vi "Perfect Number Check.vi"() -> ()   [LabVIEW 2026]
panel:
  out "Sum of Divisors":dbl
  out "Status":string
  in  "Input Number(N)":dbl
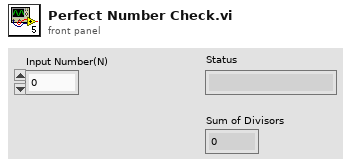
[diagram p1: front panel]
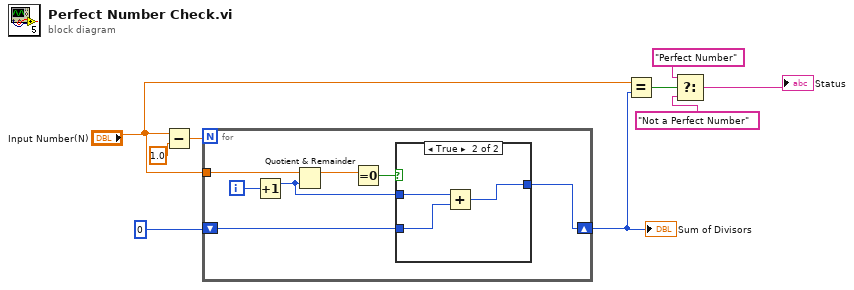
[diagram p0: block diagram]
diagram:
  n1 = Subtract(x="Input Number(N)", y=1.0) -> (x-y=w3:dbl)
  n2 = for {
    N: w3 -> [_]
    tunnel: "Input Number(N)" -> [w16]
    shift-right: [w10] -> w8
    shift-left: 0 -> [w12]
    i -> [w15]
    n3 = Increment(x=w15) -> (x+1=w11:i32)
    n4 = Quotient & Remainder(x=w16, y=w11) -> (x-y*floor(x/y)=w14:dbl)  [unwired: 1 out]
    n5 = Equal To 0?(x=w14) -> (x = 0?=w13:bool)
    n6 = case shown="True" w13 {
      tunnel: w12 -> [w17 w20]
      tunnel: w11 -> [_ w19]
      tunnel: [w17 w18] -> w10
      frame False {
      }
      frame True {
        n7 = Add(x=w19, y=w20) -> (x+y=w18:i32)
      }
    }
  }
  "Sum of Divisors" <- w8
  n8 = Equal?(x="Input Number(N)", y=w8) -> (x = y?=w7:bool)
  n9 = Select(t="Perfect Number", s=w7, f="Not a Perfect Number") -> (s? t:f=→"Status":string)
